vi "Ejemplo Case Jácome.vi"() -> ()   [LabVIEW 2026]
panel:
  out "ESTADO DEL MOTOR":string
  in  "MOTOR":bool
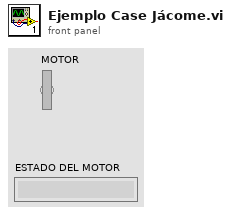
[diagram p1: front panel]
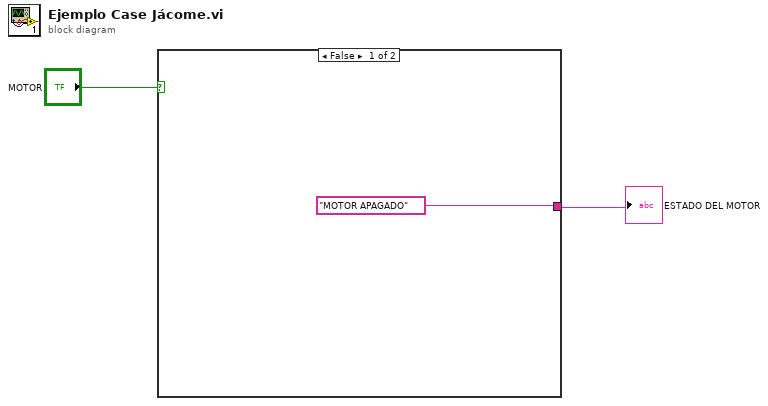
[diagram p0: block diagram]
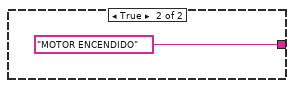
[diagram p2: hidden frame]
diagram:
  n1 = case shown="False" "MOTOR" {
    tunnel: ["MOTOR APAGADO" "MOTOR ENCENDIDO"] -> w1
    frame False {
    }
    frame True {
    }
  }
  "ESTADO DEL MOTOR" <- w1
